vi "Demo_Input.vi"(0 "Step":i32, 11 "error in":errorcluster) -> (4 "Key":u16, 15 "error out":errorcluster)   [LabVIEW 2020, in "GH_Engine.lvlib"]
doc: "Key of the demo for one demo tick (Step). Outside the listed steps: no key (0)."
uses:
  GH_Engine.lvlib
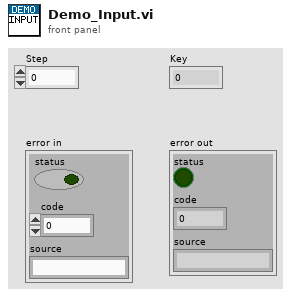
[diagram p1: front panel]
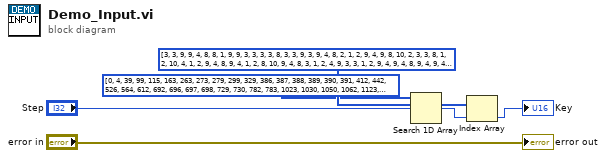
[diagram p0: block diagram]
diagram:
  n1 = Search 1D Array(1D array=i32[] [0, 4, 39, 99, 115, 163, 263, 273, 279, 299, 329, 386, 387, 388, 389, 390, 391, 412, 442, 526, 564, 612, 692, 696, 697, 698, 729, 730, 782, 783, 1023, 1030, 1050, 1062, 1123, 1124, 1145, 1155, 1159, 1163, 1173, 1203, 1223, 1245, 1255, 1259, 1262, 1276, 1277, 1281, 1341, 1365, 1493, 1642, 1646, 1668, 1669, 1729, 1749, 1774, 1775, 1776, 1807, 1808, 1868, 1928, 1948, 1954, 1964, 1994, 1995, 2028, 2029, 2050, 2060, 2064, 2068, 2078, 2108, 2128, 2220, 2409, 2549, 2550, 2586, 2604, 2605, 2640, 2654, 2702, 2722, 2877, 3023, 3131, 3147, 3167, 3197, 3213, 3306, 3322, 3342, 3364, 3394, 3422, 3438, 3458, 3468, 3472, 3473, 3474, 3475, 3479, 3539, 3667, 3837, 3838, 3901, 3911, 3917, 3937, 3967, 4031, 4124, 4201, 4273, 4277, 4278, 4299, 4309, 4313, 4317, 4327, 4350, 4351, 4591, 4597, 4708, 4890, 5198, 5202, 5203, 5207, 5208, 5209, 5210, 5211, 5216, 5246, 5310, 5371, 5375, 5397, 5398, 5458, 5462, 5501, 5641, 5692, 5796, 5912, 5913, 5934, 5944, 5948, 5952, 5962, 5992, 6012, 6037, 6038, 6059, 6069, 6073, 6077, 6087, 6117, 6137, 6346, 6507, 6547, 6569, 6579, 6580, 6582, 6603, 6635, 6679, 6699, 6816, 6844, 6856, 7001, 7005, 7051, 7052, 7073, 7083, 7087, 7091, 7101, 7131, 7151, 7154, 7448, 7536, 7537, 7538, 7569, 7570, 7630, 7697, 7730, 7731, 7752, 7762, 7766, 7770, 7780, 7810, 7830, 7869, 7870, 7871, 7931, 8035, 8036, 8057, 8067, 8071, 8075, 8085, 8115, 8211, 8410, 8491, 8495, 8515, 8540, 8541, 8542, 8573, 8574, 8634, 8654, 8766, 8767, 8788, 8798, 8802, 8806, 8816, 8846, 9034, 9035, 9056, 9066, 9070, 9074, 9084, 9114, 9126, 9136, 9147, 9157, 9176, 9197, 9216, 9236, 9299, 9300, 9301, 9361, 9393, 9433, 9502, 9506, 9507, 9528, 9538, 9542, 9546, 9556, 9586, 9690, 9734, 9756, 9766, 9770, 9773, 9803, 9804, 9880, 9981, 9997, 10017, 10047, 10051, 10230, 10412, 10428, 10448, 10478, 10515, 10529, 10534, 10541, 10585, 10658, 10731, 10732, 10742, 10802, 10893, 10897, 10898, 10919, 10929, 10933, 10937, 10947, 10977, 11161, 11165, 11185, 11206, 11244, 11245, 11275, 11276, 11277, 11388, 11389, 11410, 11420, 11424, 11428, 11438, 11468, 11572, 11696, 11804, 11905, 11921, 11941, 11971, 12152, 12189, 12340, 12341, 12381, 12488, 12489, 12510, 12520, 12524, 12528, 12538, 12568, 12588, 12730, 12925, 12992, 12998, 13018, 13119, 13259, 13275, 13295, 13325, 13457, 13477, 13642, 13646, 13666, 13687, 13835, 13836, 13857, 13867, 13871, 13875, 13885, 13915, 14019, 14199, 14200, 14201, 14232, 14233, 14293, 14297, 14433, 14466, 14467, 14488, 14498, 14502, 14506, 14516, 14546, 14726, 14727, 14748, 14758, 14762, 14766, 14776, 14806, 14826, 14910, 14971, 14972, 14973, 14994, 15328] ("Demo steps"), element="Step") -> (index of element=w5:i32)  [unwired: 1 in]
  n2 = Index Array(array=u16[] [3, 3, 9, 9, 4, 8, 8, 1, 9, 9, 3, 3, 3, 3, 8, 3, 3, 9, 3, 9, 4, 8, 2, 1, 2, 9, 4, 9, 8, 10, 2, 3, 3, 8, 1, 2, 10, 4, 1, 2, 9, 4, 8, 9, 4, 1, 2, 8, 10, 9, 4, 8, 3, 1, 2, 4, 9, 3, 3, 1, 2, 9, 4, 9, 4, 8, 9, 4, 9, 4, 8, 1, 2, 10, 3, 1, 2, 9, 3, 3, 8, 1, 10, 8, 9, 3, 1, 4, 9, 4, 4, 2, 8, 8, 1, 9, 3, 8, 8, 9, 9, 9, 4, 8, 9, 8, 8, 9, 10, 8, 4, 9, 4, 8, 3, 4, 8, 1, 9, 9, 3, 8, 4, 8, 2, 1, 2, 10, 3, 1, 2, 9, 8, 10, 2, 3, 10, 8, 1, 2, 8, 4, 4, 3, 8, 10, 9, 3, 4, 1, 2, 4, 9, 3, 3, 8, 9, 4, 8, 1, 2, 10, 3, 1, 2, 9, 3, 3, 1, 2, 10, 4, 1, 2, 9, 3, 3, 4, 8, 8, 10, 3, 1, 9, 9, 4, 2, 4, 8, 3, 8, 1, 2, 1, 2, 10, 4, 1, 2, 9, 3, 3, 8, 8, 1, 2, 9, 4, 9, 4, 8, 1, 2, 10, 3, 1, 2, 9, 3, 3, 3, 3, 9, 3, 1, 2, 10, 4, 1, 2, 9, 4, 8, 8, 1, 2, 4, 1, 2, 9, 4, 9, 3, 3, 1, 2, 10, 4, 1, 2, 9, 4, 1, 2, 10, 3, 1, 2, 9, 4, 8, 3, 1, 9, 9, 8, 3, 3, 3, 3, 9, 3, 4, 4, 2, 1, 2, 10, 3, 1, 2, 9, 4, 8, 8, 9, 4, 1, 2, 4, 3, 8, 8, 1, 9, 3, 3, 2, 8, 1, 9, 3, 8, 3, 9, 3, 3, 4, 4, 9, 9, 4, 2, 1, 2, 10, 3, 1, 2, 9, 4, 1, 2, 4, 8, 3, 9, 4, 3, 4, 1, 2, 10, 3, 1, 2, 9, 4, 8, 3, 8, 8, 1, 9, 3, 2, 8, 10, 8, 2, 1, 2, 10, 4, 1, 2, 9, 3, 3, 8, 4, 1, 2, 4, 8, 8, 1, 9, 4, 2, 4, 1, 2, 4, 8, 1, 2, 10, 3, 1, 2, 9, 4, 8, 1, 2, 9, 4, 9, 3, 3, 8, 1, 2, 10, 4, 1, 2, 9, 4, 1, 2, 10, 3, 1, 2, 9, 3, 3, 8, 3, 3, 3, 9, 4] ("Demo keys"), index=w5) -> (element=→"Key":u16)
  "error out" <- "error in"
